vi "nominal teststand model options dialog.vi"(10 "config in":T1, 11 "Sequence Context":refnum<k7>) -> (2 "config out":T1, 4 "error out":errorcluster)   [LabVIEW 2020, in "nominal teststand model sequence support.lvlib"]
doc: "This VI is an example of a dialog box that is modal to the TestStand main application window using the TestStand Utility VIs. A modal dialog prevents the user from interacting with the TestStand Application until the modal dialog is dismissed."
uses:
  nominal teststand model sequence support.lvlib
  <vilib>/addons/TestStand/_TSUtility.llb/TestStand - Start Modal Dialog (Sequence Context).vi
  <vilib>/addons/TestStand/_TSUtility.llb/TestStand - End Modal Dialog (Sequence Context).vi
panel:
  in  "Nominal Core API Key":string
  in  "Asset prefix":string
  in  "Dataset Name (optional)":string
  in  "Asset RID":string
  in  "Dataset RID":string
  out "Explanation":string
  in  "Mode":T2(ring)
  in  "save":bool
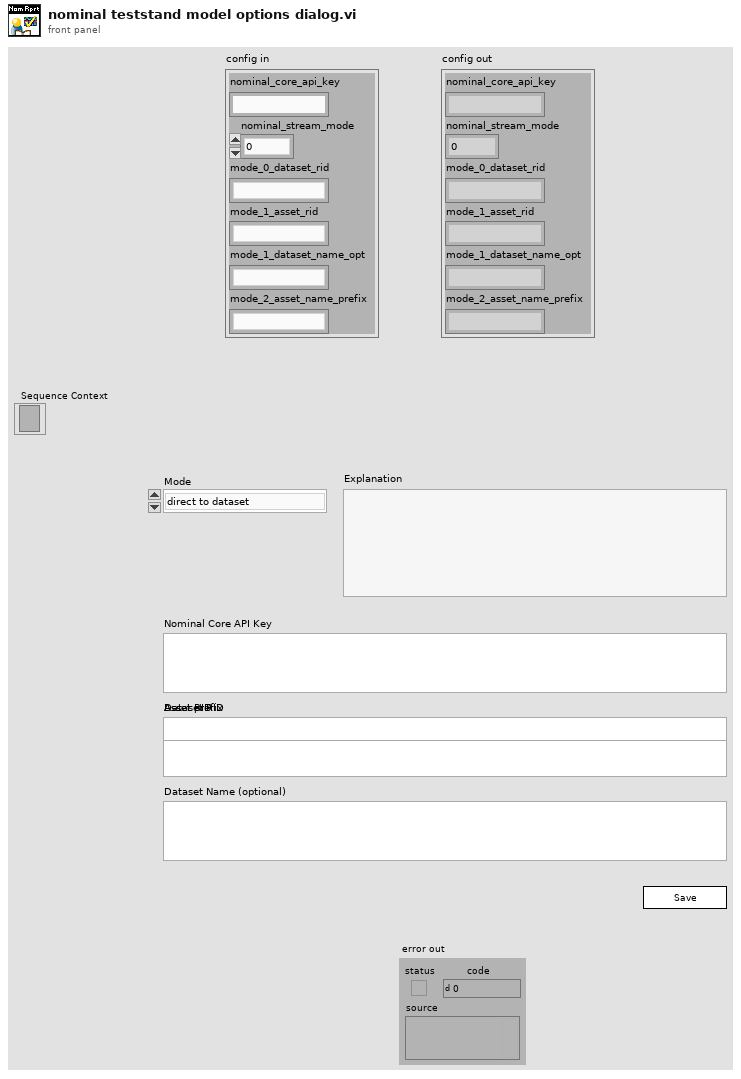
[diagram p1: front panel]
types:
  T1 = cluster{"nominal_core_api_key":string, "nominal_stream_mode":u8, "mode_0_dataset_rid":string, "mode_1_asset_rid":string, "mode_1_dataset_name_opt":string, "mode_2_asset_name_prefix":string}
  T2 = enum16{"direct to dataset", "stream to asset", "generate asset per test"}
  T3 = cluster{"Dataset RID":refnum<vi>, "Asset RID":refnum<vi>, "Dataset Name (optional)":refnum<vi>, "Asset prefix":refnum<vi>}
  T4 = cluster{"mode_0_dataset_rid":bool, "mode_1_asset_rid":bool, "mode_1_dataset_name_opt":bool, "mode_2_asset_name_prefix":bool}
  T5 = cluster{"mode_0_dataset_rid":string, "mode_1_asset_rid":string, "mode_1_dataset_name_opt":string, "mode_2_asset_name_prefix":string}
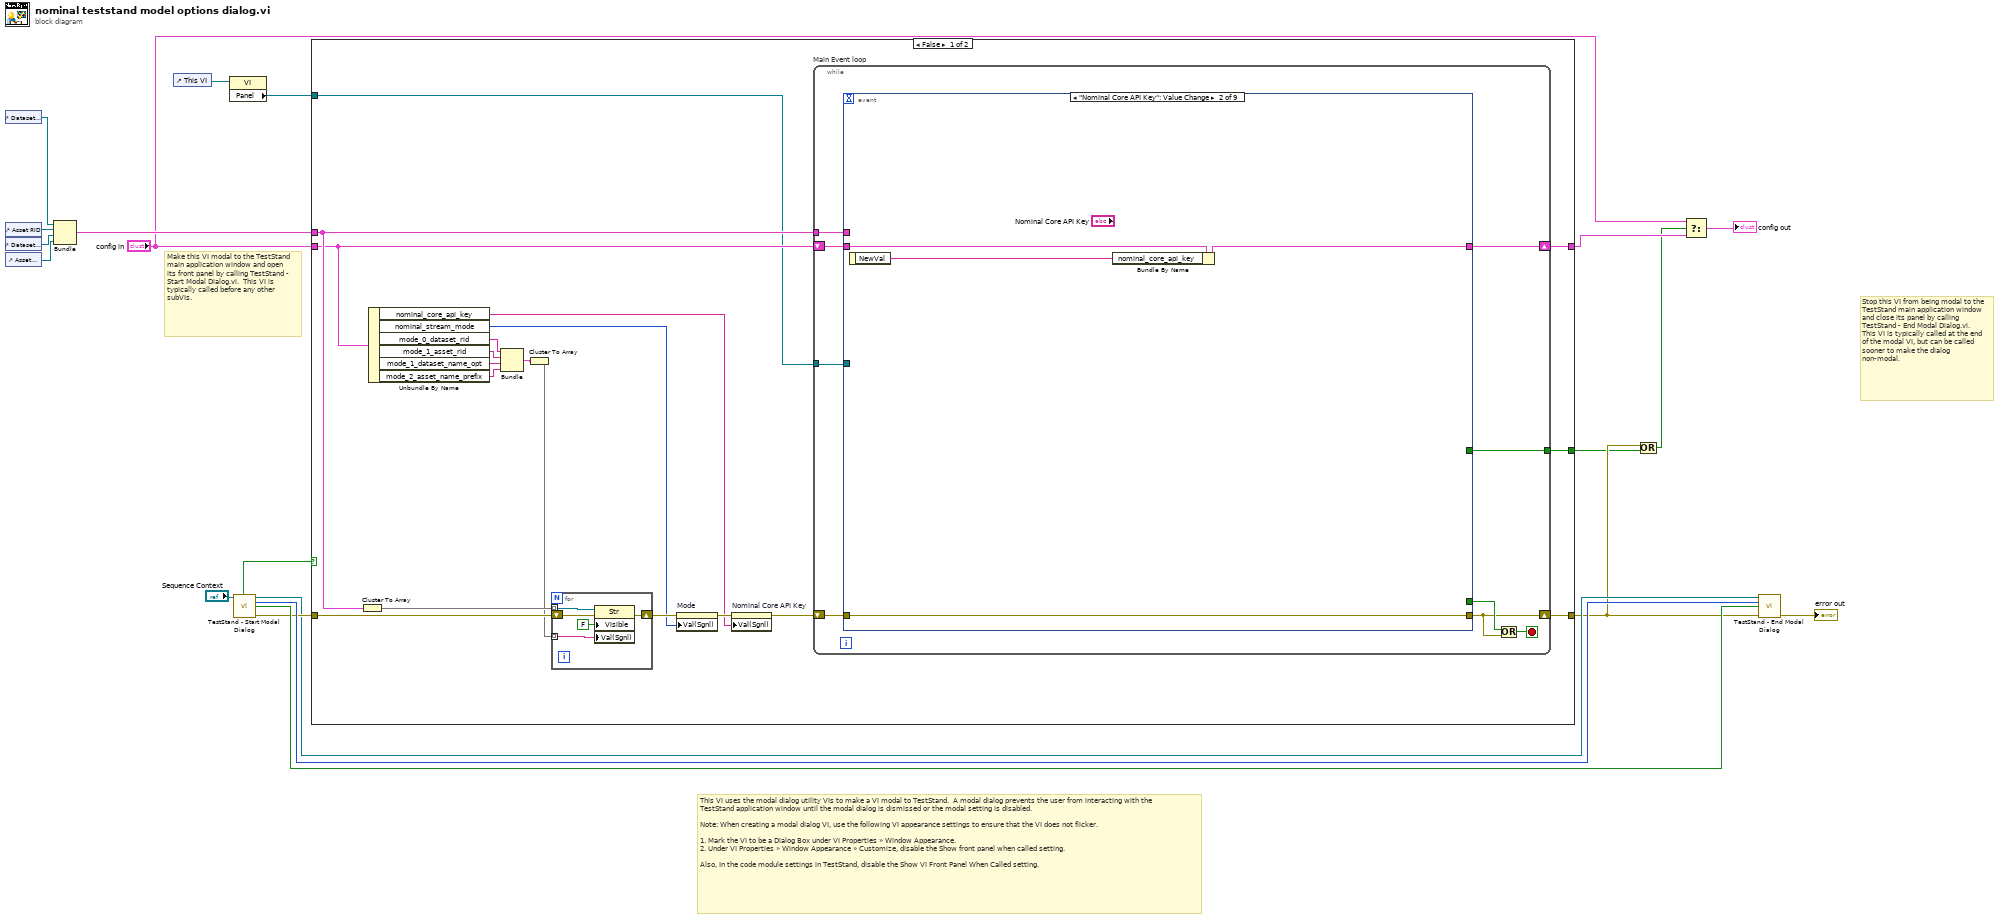
[diagram p0: block diagram]
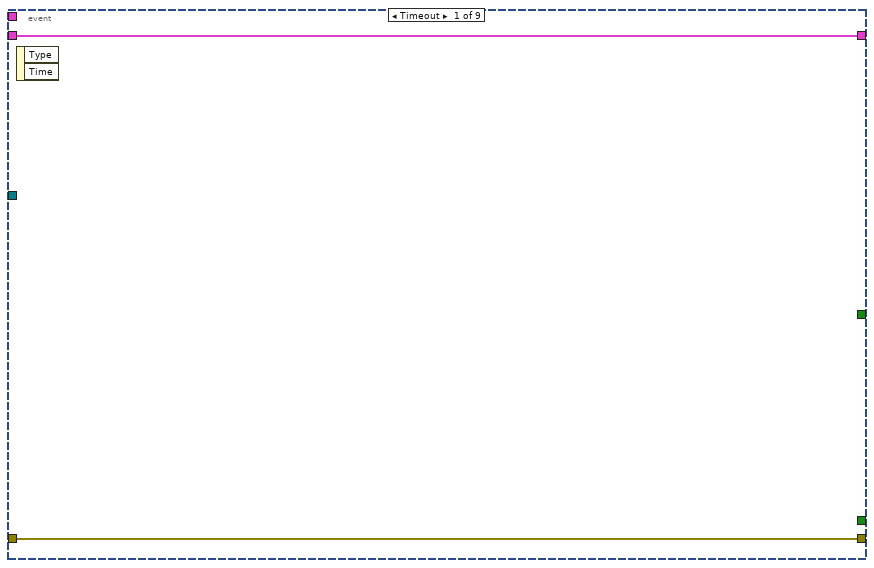
[diagram p2: hidden frame]
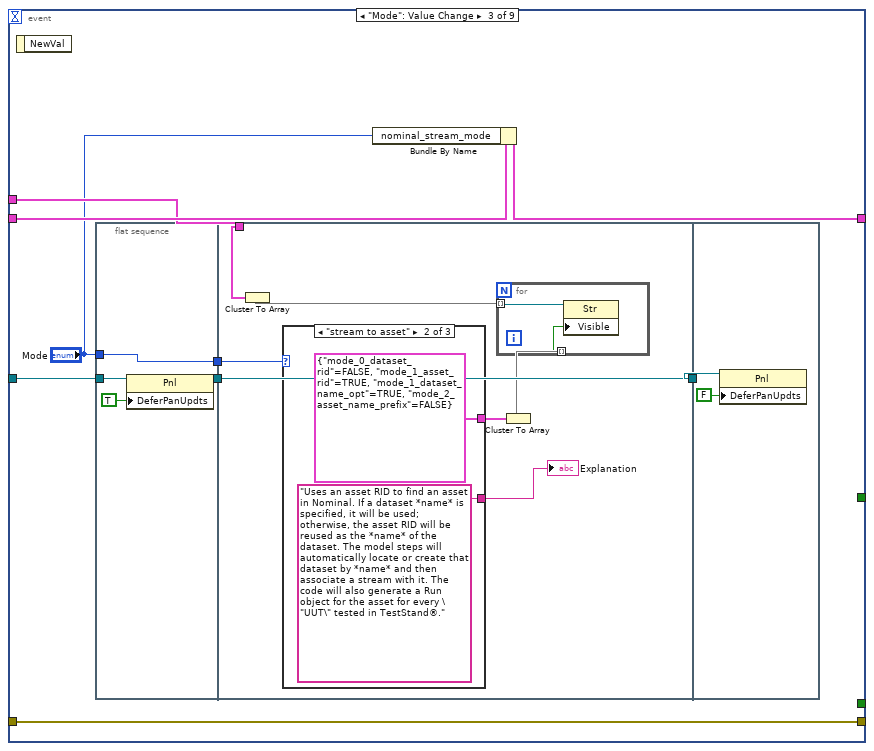
[diagram p3: hidden frame]
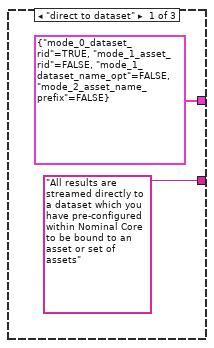
[diagram p4: hidden frame]
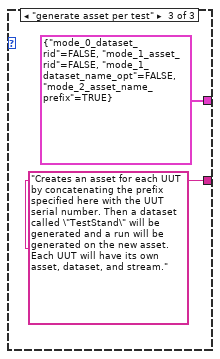
[diagram p5: hidden frame]
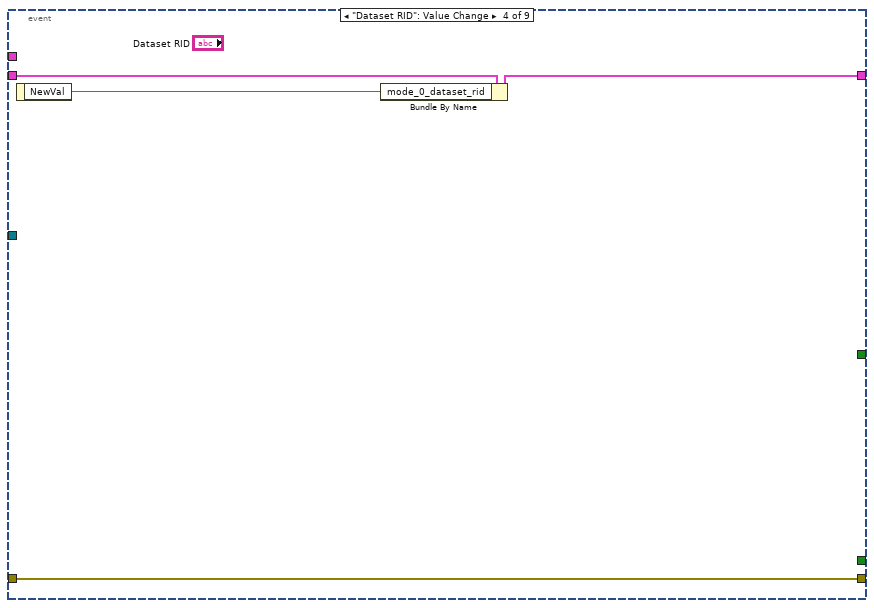
[diagram p6: hidden frame]
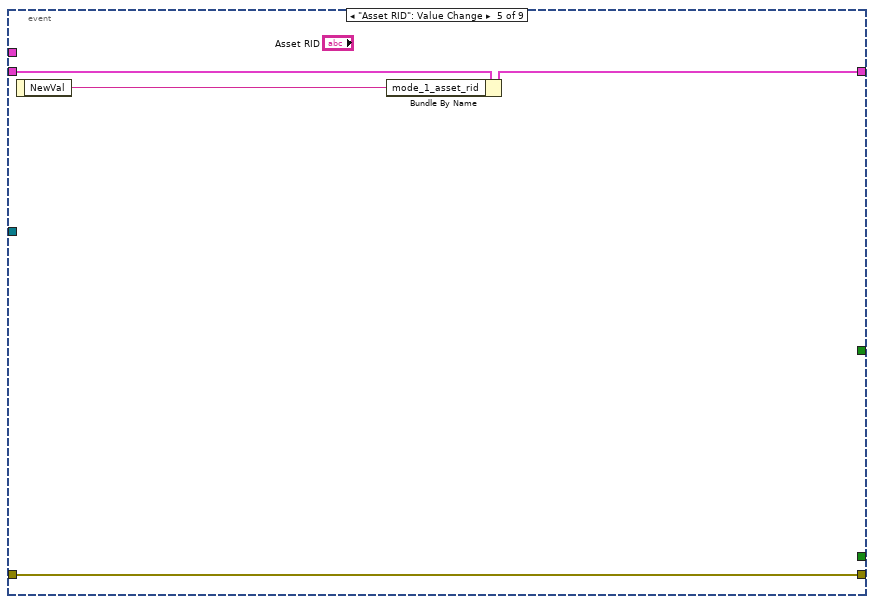
[diagram p7: hidden frame]
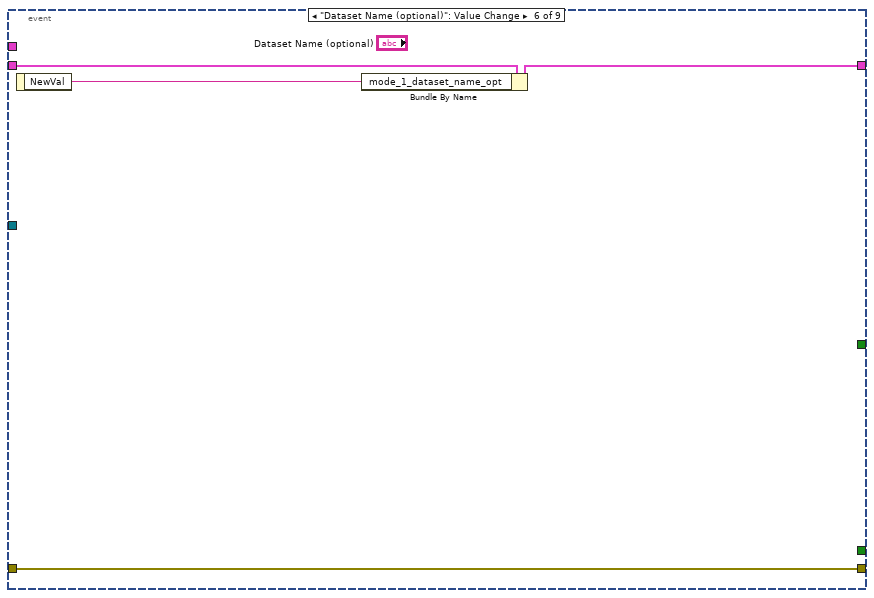
[diagram p8: hidden frame]
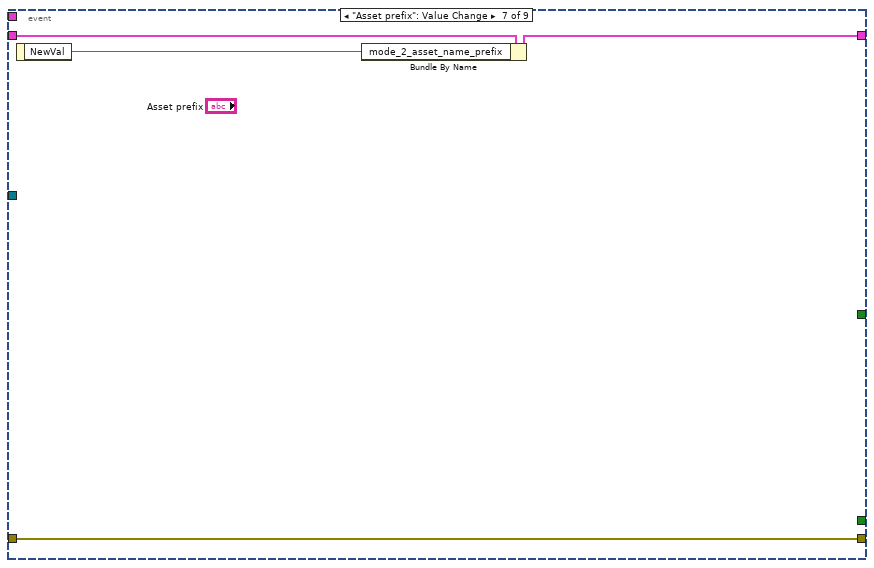
[diagram p9: hidden frame]
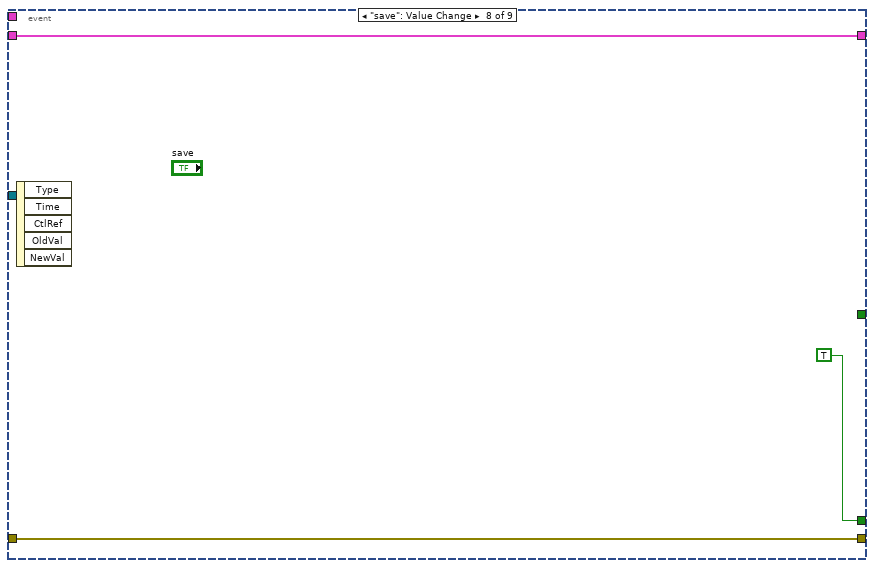
[diagram p10: hidden frame]
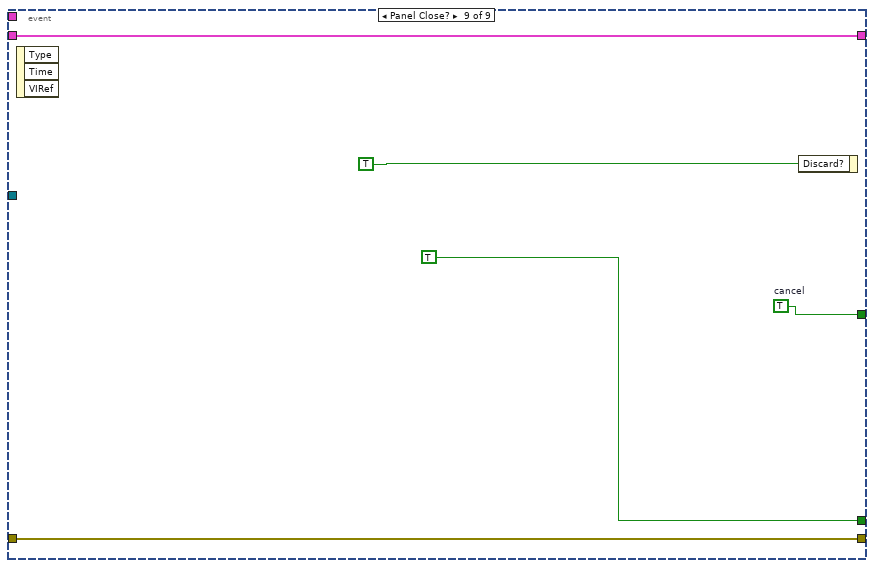
[diagram p11: hidden frame]
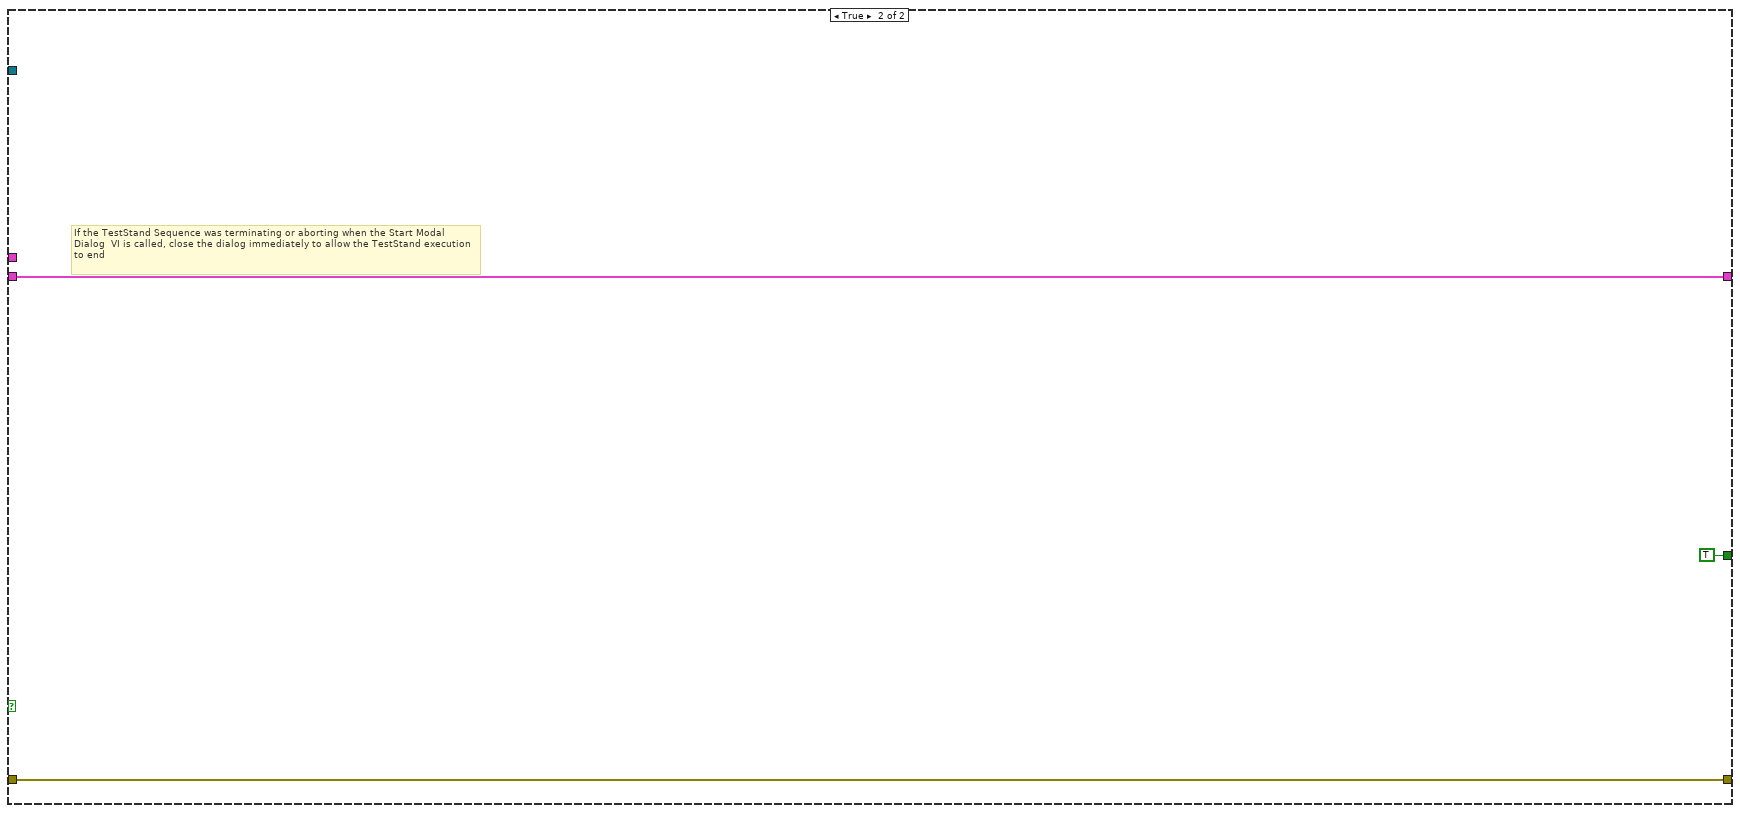
[diagram p12: hidden frame]
diagram:
  # "Make this VI modal to the TestStand main application window and open its front panel by calling TestStand - Start Modal Dialog.vi.  This VI is typically called before any other subVIs."
  # "Stop this VI from being modal to the TestStand main application window and close its panel by calling TestStand - End Modal Dialog.vi.  This VI is typically called at the end of the modal VI, but can be called sooner to make the dialog non-modal."
  # "This VI uses the modal dialog utility VIs to make a VI modal to TestStand.  A modal dialog prevents the user from interacting with the TestStand application window until the modal dialog is dismissed or the modal setting is disabled.\n\nNote: When creating a modal dialog VI, use the following VI appearance settings to ensure that the VI does not flicker.\n\n1. Mark the VI to be a Dialog Box under VI Properties » Window Appearance.\n2. Under VI Properties » Window Appearance » Customize, disable the Show front panel when called setting.\n\nAlso, In the code module settings in TestStand, disable the Show VI Front Panel When Called setting."
  n1 = control-ref of="Dataset RID"() -> (w13:refnum<vi>)
  n2 = control-ref of="Asset RID"() -> (w12:refnum<vi>)
  n3 = control-ref of="Dataset Name (optional)"() -> (w11:refnum<vi>)
  n4 = control-ref of="Asset prefix"() -> (w10:refnum<vi>)
  n5 = Bundle("Dataset RID"=w13, "Asset RID"=w12, "Dataset Name (optional)"=w11, "Asset prefix"=w10) -> (w9:T3)  [unwired: 1 in]
  n6 = control-ref of="This VI"() -> (w4:refnum<vi>)
  n7 = property class="VI"(reference=w4) -> ("Panel"=w3:refnum<vi>)  [unwired: 1 in, 2 out]
  n8 = call-poly <vilib>:"TestStand - Start Modal Dialog.vi"("Sequence Context In"="Sequence Context") -> ("Sequence Context Out"=w14:refnum<k7>, "Modal ID"=w18:i32, "VI Originally Open"=w17:bool, "Should Abort"=w19:bool, "error out"=w16:errorcluster)  [unwired: 2 in, 8 out]
  n9 = case shown="False" w19 {
    tunnel: w16 -> [w39 w116]
    tunnel: [w38 w116] -> w8
    tunnel: w9 -> [w36 _]
    tunnel: "config in" -> [w33 w115]
    tunnel: [w34 w115] -> w6
    tunnel: w3 -> [w26 _]
    tunnel: [w21 TRUE ("cancel")] -> w1
    frame False {
      n10 = Cluster To Array(cluster=w36) -> (array=w35:refnum<vi>[])
      n11 = Unbundle By Name(w33) -> ("nominal_core_api_key"=w22:string, "nominal_stream_mode"=w23:u8, "mode_0_dataset_rid"=w32:string, "mode_1_asset_rid"=w31:string, "mode_1_dataset_name_opt"=w30:string, "mode_2_asset_name_prefix"=w29:string)
      n12 = Bundle("mode_0_dataset_rid"=w32, "mode_1_asset_rid"=w31, "mode_1_dataset_name_opt"=w30, "mode_2_asset_name_prefix"=w29) -> (w28:T5)  [unwired: 1 in]
      n13 = Cluster To Array(cluster=w28) -> (array=w27:string[])
      n14 = for {
        tunnel: w35 -> [w42] mode=indexing
        shift-right: [w43] -> w37
        shift-left: w39 -> [w44]
        tunnel: w27 -> [w40] mode=indexing
        n15 = property class="Str"(reference=w42, error in=w44, "Visible"=FALSE, "Val(Sgnl)"=w40) -> (error out=w43:errorcluster)  [unwired: 1 out]
      }
      n16 = property on="Mode" class="Enum (strict)"(error in=w37, "Val(Sgnl)"=w23) -> (error out=w25:errorcluster)  [unwired: 1 in, 1 out]
      n17 = property on="Nominal Core API Key" class="Str"(error in=w25, "Val(Sgnl)"=w22) -> (error out=w24:errorcluster)  [unwired: 1 in, 1 out]
      n18 = while "Main Event loop" {
        tunnel: w36 -> [w51]
        shift-right: [w49] -> w34
        shift-left: w33 -> [w50]
        shift-right: [w47] -> w38
        shift-left: w24 -> [w52]
        tunnel: w26 -> [w46]
        tunnel: [w45] -> w21
        stop <- w48 stop-if-true
        n19 = event shown="[1] \"Nominal Core API Key\": Value Change" {
          selector: _ -> [_ _ _ _ _ _ _ _ _]
          dyn-events: _ -> [_ _ _ _ _ _ _ _ _]
          timeout: _ -> [_ _ _ _ _ _ _ _ _]
          tunnel: [_ _ _ _ _ _ _ TRUE ("NewVal") TRUE ("NewVal")] -> w53
          tunnel: [w54 w59 w68 w93 w97 w101 w105 w108 w110] -> w47
          tunnel: w52 -> [w54 w59 w68 w93 w97 w101 w105 w108 w110]
          tunnel: w51 -> [_ _ w63 _ _ _ _ _ _]
          tunnel: w50 -> [w55 w58 w67 w92 w96 w100 w104 w106 w111]
          tunnel: [w55 w57 w61 w91 w95 w99 w103 w106 w111] -> w49
          tunnel: w46 -> [_ _ w66 _ _ _ _ _ _]
          tunnel: [_ _ _ _ _ _ _ _ w109] -> w45
          event Timeout {
            n20 = event-data() -> ()  [unwired: 1 in, 2 out]
          }
          event "Nominal Core API Key": Value Change {
            n21 = event-data() -> ("NewVal"=w56:string)  [unwired: 1 in]
            n22 = Bundle By Name(cluster=w58, "nominal_core_api_key"=w56) -> (w57:T1)
          }
          event "Mode": Value Change {
            n23 = event-data() -> ()  [unwired: 1 in, 1 out]
            n24 = flat-sequence {
              tunnel: w66 -> [w71]
              tunnel: [w70] -> w64
              tunnel: [w69] -> w62
              tunnel: "Mode" -> [w69]
              tunnel: [w79] -> w65
              tunnel: w64 -> [w79]
              tunnel: w63 -> [w78]
              tunnel: w62 -> [w73]
              tunnel: w65 -> [w88]
              frame #0 {
                n25 = property class="Pnl"(reference=w71, "DeferPanUpdts"=TRUE ("Defer Panel Updates")) -> (reference out=w70:refnum<vi>)  [unwired: 1 in, 1 out]
              }
              frame #1 {
                n26 = Cluster To Array(cluster=w78) -> (array=w77:refnum<vi>[])
                n27 = case shown="\"stream to asset\"" w73 {
                  tunnel: [T4 {"mode_0_dataset_rid"=TRUE, "mode_1_asset_rid"=FALSE, "mode_1_dataset_name_opt"=FALSE, "mode_2_asset_name_prefix"=FALSE} ("mode visibility") T4 {"mode_0_dataset_rid"=FALSE, "mode_1_asset_rid"=TRUE, "mode_1_dataset_name_opt"=TRUE, "mode_2_asset_name_prefix"=FALSE} ("mode visibility") T4 {"mode_0_dataset_rid"=FALSE, "mode_1_asset_rid"=FALSE, "mode_1_dataset_name_opt"=FALSE, "mode_2_asset_name_prefix"=TRUE} ("mode visibility")] -> w76
                  tunnel: ["All results are streamed directly to a dataset which you have pre-configured within Nominal Core to be bound to an asset or set of assets" "Uses an asset RID to find an asset in Nominal. If a dataset *name* is specified, it will be used; otherwise, the asset RID will be reused as the *name* of the dataset. The model steps will automatically locate or create that dataset by *name* and then associate a stream with it. The code will also generate a Run object for the asset for every \"UUT\" tested in TestStand®." "Creates an asset for each UUT by concatenating the prefix specified here with the UUT serial number. Then a dataset called \"TestStand\" will be generated and a run will be generated on the new asset. Each UUT will have its own asset, dataset, and stream."] -> w74
                  frame "direct to dataset" {
                  }
                  frame "stream to asset" {
                  }
                  frame "generate asset per test" {
                  }
                }
                "Explanation" <- w74
                n28 = Cluster To Array(cluster=w76) -> (array=w75:bool[])
                n29 = for {
                  tunnel: w77 -> [w87] mode=indexing
                  tunnel: w75 -> [w86] mode=indexing
                  n30 = property class="Str"(reference=w87, "Visible"=w86) -> ()  [unwired: 1 in, 2 out]
                }
              }
              frame #2 {
                n31 = property class="Pnl"(reference=w88, "DeferPanUpdts"=FALSE ("Defer Panel Updates")) -> ()  [unwired: 1 in, 2 out]
              }
            }
            n32 = Bundle By Name(cluster=w67, "nominal_stream_mode"="Mode") -> (w61:T1)
          }
          event "Dataset RID": Value Change {
            n33 = event-data() -> ("NewVal"=w90:string)  [unwired: 1 in]
            n34 = Bundle By Name(cluster=w92, "mode_0_dataset_rid"=w90) -> (w91:T1)
          }
          event "Asset RID": Value Change {
            n35 = event-data() -> ("NewVal"=w94:string)  [unwired: 1 in]
            n36 = Bundle By Name(cluster=w96, "mode_1_asset_rid"=w94) -> (w95:T1)
          }
          event "Dataset Name (optional)": Value Change {
            n37 = event-data() -> ("NewVal"=w98:string)  [unwired: 1 in]
            n38 = Bundle By Name(cluster=w100, "mode_1_dataset_name_opt"=w98) -> (w99:T1)
          }
          event "Asset prefix": Value Change {
            n39 = event-data() -> ("NewVal"=w102:string)  [unwired: 1 in]
            n40 = Bundle By Name(cluster=w104, "mode_2_asset_name_prefix"=w102) -> (w103:T1)
          }
          event "save": Value Change {
            n41 = event-data() -> ()  [unwired: 1 in, 5 out]
          }
          event Panel Close? {
            w109 = TRUE  # cancel
            n42 = event-data() -> ()  [unwired: 1 in, 3 out]
            n43 = event-data("Discard?"=TRUE ("NewVal")) -> ()  [unwired: 1 in, 1 out]
          }
        }
        n44 = Or(x=w53, y=w47) -> (x .or. y?=w48:bool)
      }
    }
    frame True {
      # "If the TestStand Sequence was terminating or aborting when the Start Modal Dialog  VI is called, close the dialog immediately to allow the TestStand execution to end"
    }
  }
  n45 = Or(x=w8, y=w1) -> (x .or. y?=w2:bool)
  n46 = Select(t="config in", s=w2, f=w6) -> (s? t:f=→"config out":T1)
  n47 = call-poly <vilib>:"TestStand - End Modal Dialog.vi"("Sequence Context In"=w14, "Modal ID"=w18, "VI Originally Open"=w17, "error in (no error)"=w8) -> ("error out"=→"error out":errorcluster)  [unwired: 1 in, 10 out]
